vi "Overwrite Dialog.vi"(8 "error in (no error)":errorcluster, 11 "Path":path) -> (0 "error out":errorcluster, 3 "Cancelled?":bool)   [LabVIEW 2020, in "Caraya.lvlib" / "Basic Test Manager.lvclass"]
uses:
  Basic Test Manager.lvclass
panel:
  out "String":string
  in  "Cancel":bool
  in  "Overwrite":bool
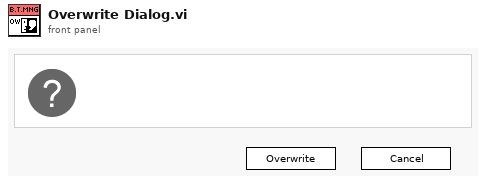
[diagram p1: front panel]
types:
  T1 = enum32{"Invalid", "Standard", "Closed", "Hidden", "Minimized", "Maximized"}
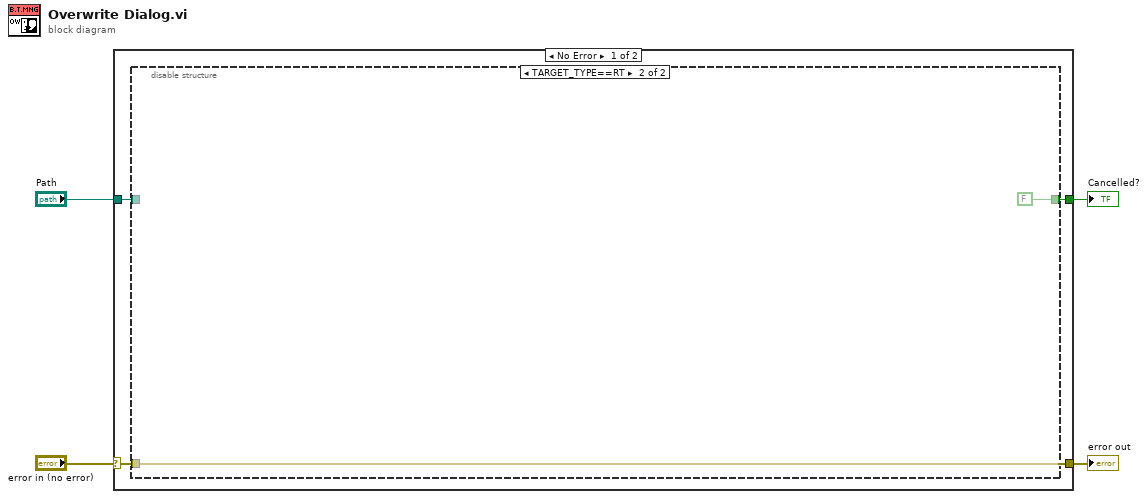
[diagram p0: block diagram]
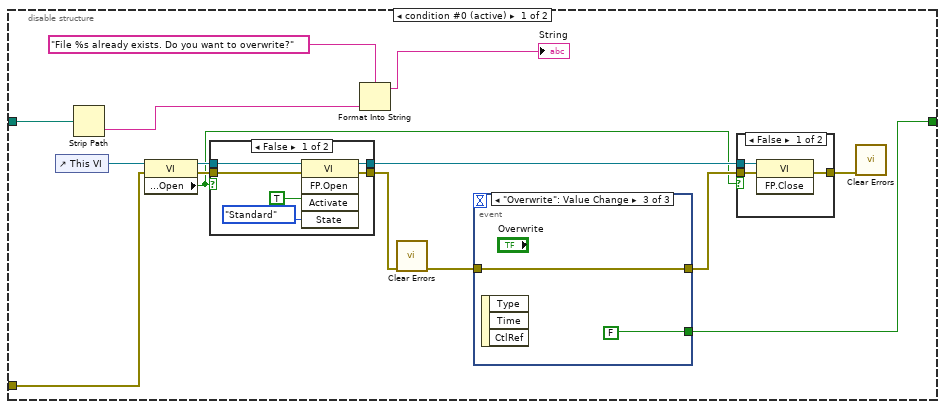
[diagram p2: hidden frame]
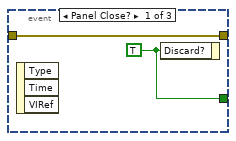
[diagram p5: hidden frame]
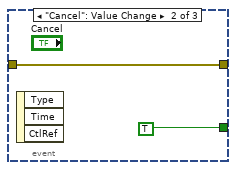
[diagram p6: hidden frame]
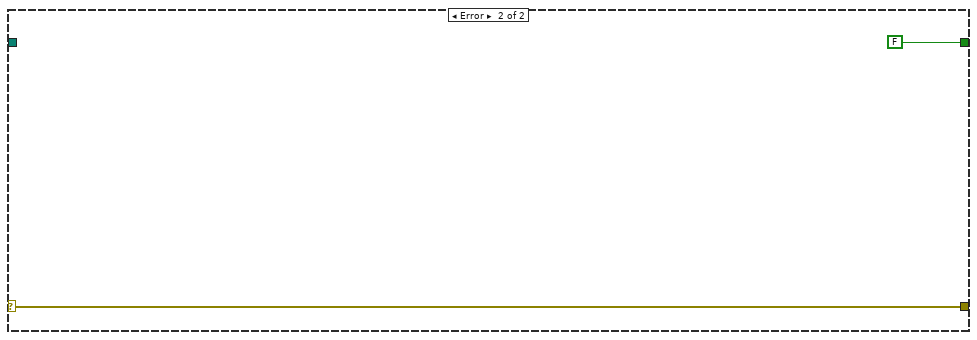
[diagram p7: hidden frame]
diagram:
  n1 = case shown="No Error" "error in (no error)" {
    selector: "error in (no error)" -> [w7 w43]
    tunnel: [w7 w43] -> w3
    tunnel: [w5 FALSE ("Discard?")] -> w1
    tunnel: "Path" -> [w6 _]
    frame No Error {
      n2 = disable-structure shown="TARGET_TYPE==RT" {
        disable-tunnel: w7 -> [w13 _]
        disable-tunnel: w6 -> [w12 _]
        disable-tunnel: [w8 FALSE ("Discard?")] -> w5
        frame condition #0 (active) {
          n3 = control-ref of="This VI"() -> (w22:refnum<vi>)
          n4 = Strip Path(path=w12) -> (name=w10:string)  [unwired: 1 out]
          n5 = property class="VI"(reference=w22, error in=w13) -> (reference out=w20:refnum<vi>, error out=w21:errorcluster, "Front Panel.Open"=w14:bool)
          n6 = case shown="False" w14 {
            tunnel: [w30 w34] -> w19
            tunnel: w21 -> [w29 w34]
            tunnel: w20 -> [w28 w33]
            tunnel: [w27 w33] -> w16
            frame False {
              n7 = invoke class="VI" method="FP.Open"(reference=w28, error in=w29, "Activate"=TRUE, "State"=T1."Standard") -> (reference out=w27:refnum<vi>, error out=w30:errorcluster)  [unwired: 1 in, 3 out]
            }
            frame True {
            }
          }
          n8 = Format Into String(format string="File %s already exists. Do you want to overwrite?" ("String"), w10) -> (resulting string=→"String":string)  [unwired: 2 in, 1 out]
          n9 = call <vilib>:"Clear Errors.vi"("error in (no error)"=w19) -> ("error out"=w18:errorcluster)  [unwired: 5 in, 1 out]
          n10 = event shown="[2] \"Overwrite\": Value Change" {
            selector: _ -> [_ _ _]
            dyn-events: _ -> [_ _ _]
            timeout: _ -> [_ _ _]
            tunnel: w18 -> [w36 w38 w40]
            tunnel: [w36 w38 w40] -> w15
            tunnel: [w35 TRUE ("Discard?") FALSE ("Discard?")] -> w8
            event Panel Close? {
              w35 = TRUE ("Discard?")
              n11 = event-data() -> ()  [unwired: 1 in, 3 out]
              n12 = event-data("Discard?"=w35) -> ()  [unwired: 1 in, 1 out]
            }
            event "Cancel": Value Change {
              n13 = event-data() -> ()  [unwired: 1 in, 3 out]
            }
            event "Overwrite": Value Change {
              n14 = event-data() -> ()  [unwired: 1 in, 3 out]
            }
          }
          n15 = case shown="False" w14 {
            tunnel: [w25 w26] -> w17
            tunnel: w15 -> [w24 w26]
            tunnel: w16 -> [w23 _]
            frame False {
              n16 = invoke class="VI" method="FP.Close"(reference=w23, error in=w24) -> (error out=w25:errorcluster)  [unwired: 1 in, 2 out]
            }
            frame True {
            }
          }
          n17 = call <vilib>:"Clear Errors.vi"("error in (no error)"=w17) -> ()  [unwired: 5 in, 2 out]
        }
        frame condition #1 {
        }
      }
    }
    frame Error {
    }
  }
  "error out" <- w3
  "Cancelled?" <- w1
